vi "Setup.vi"(4 "Exit on Error / V / H (T)":bool=TRUE, 5 "Description":string, 6 "Arguments (From Args)":string[](array[string]), 7 "Name":string, 8 "error in (no error)":errorcluster, 9 "Version":string, 11 "Arguments":T1[](array[typedef]) {"Number" items=["? One or none"=0, "* Any"=-1, "+ At least one"=-2]}) -> (0 "error out":errorcluster, 2 "Output":string, 3 "LV Argument Parser out":refnum<class "LV Argument Parser.lvclass">)   [LabVIEW 2020, in "LV ArgParse.lvlib" / "LV Argument Parser.lvclass"]
uses:
  LV Argument Parser.lvclass
  Argument Definition.ctl
  Program Info.ctl
  LV Argument Parser.lvclass/LV Argument Parser.ctl
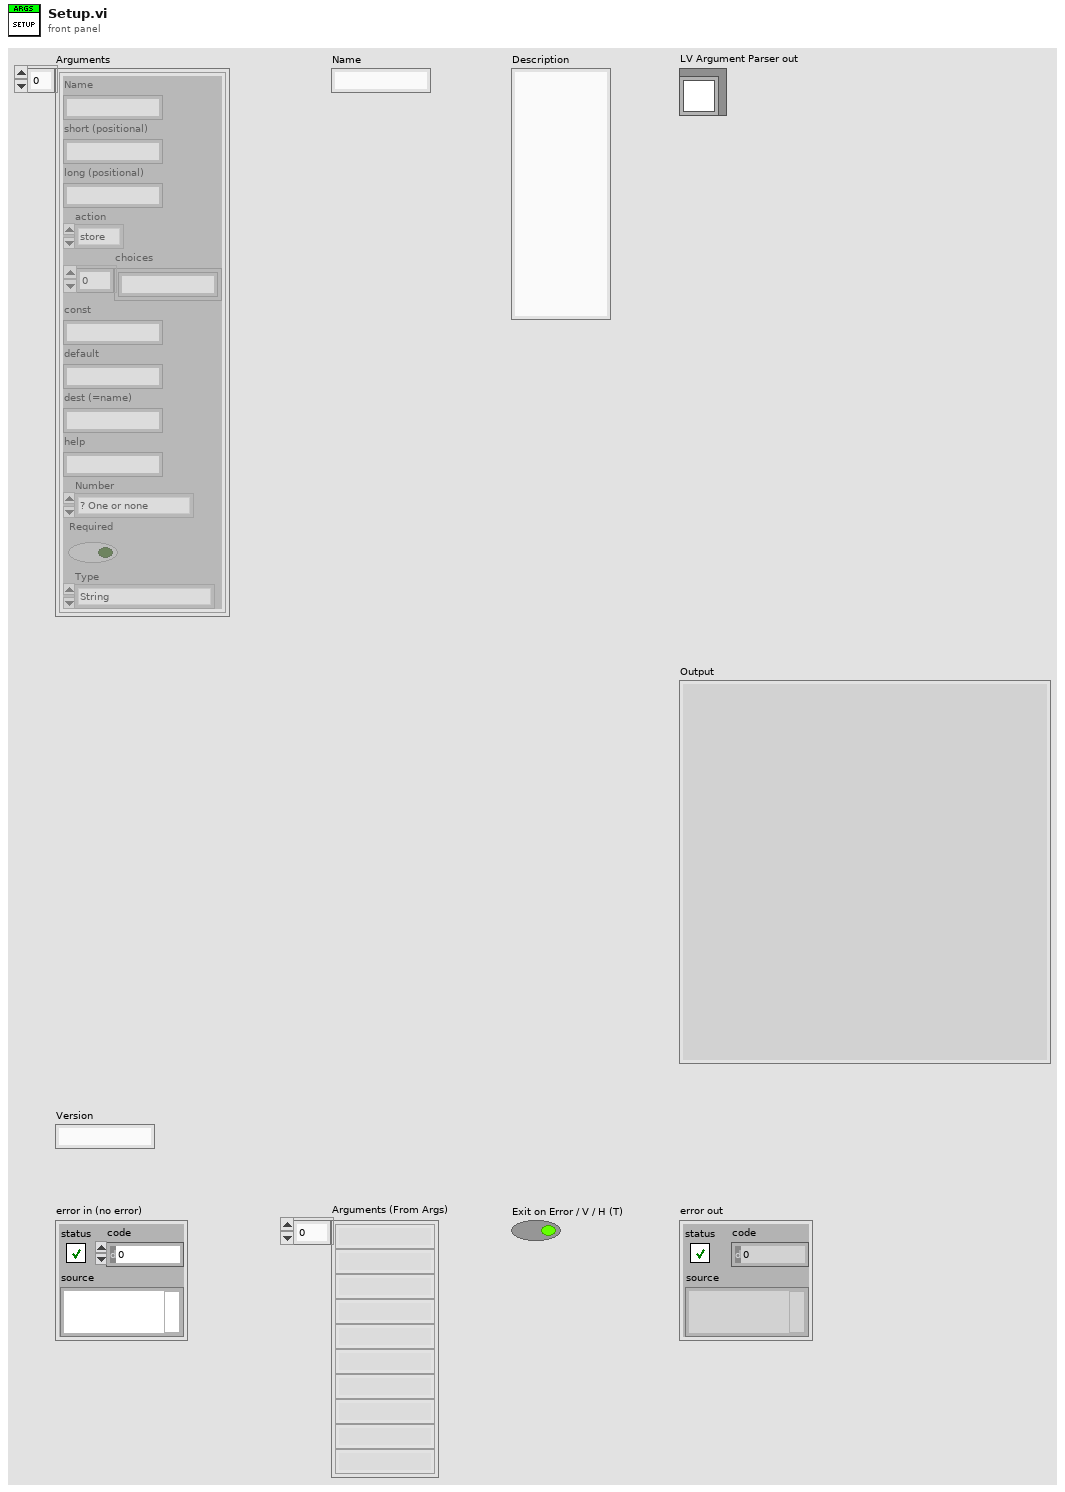
[diagram p1: front panel]
types:
  T1 = typedef "LV ArgParse.lvlib/LV Argument Parser.lvclass/Argument Definition.ctl" = cluster{"Name":string, "short (positional)":string, "long (positional)":string, "action":enum16{"store", "store-const", "store-false", "store-true", "append", "append-const", "count", "help", "version"}, "choices":string[], "const":string, "default":string, "dest (=name)":string, "help":string, "Number":i32, "Required":bool, "Type":enum16{"String", "Int", "UInt", "Float", "Bool", "Date", "Path"}}
  T2 = typedef "LV ArgParse.lvlib/LV Argument Parser.lvclass/Program Info.ctl" = cluster{"Name":string, "Description":string, "Version":string}
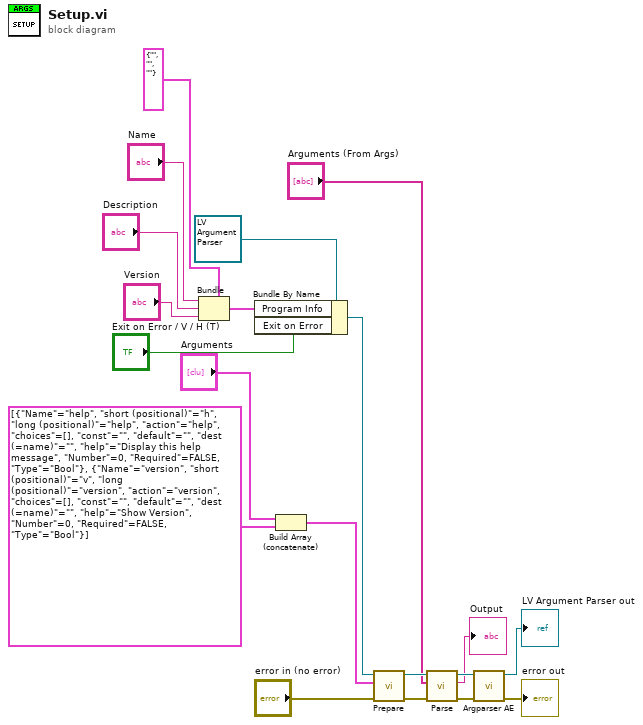
[diagram p0: block diagram]
diagram:
  n1 = Bundle(cluster=T2 {"Name"="", "Description"="", "Version"=""} ("Program Info"), "Name"="Name", "Description"="Description", "Version"="Version") -> (w13:T2)
  n2 = Bundle By Name(cluster=refnum<class "LV Argument Parser.lvclass"> refnum ("LV Argument Parser in"), "Program Info"=w13, "Exit on Error"="Exit on Error / V / H (T)") -> (w14:refnum<class "LV Argument Parser.lvclass">)
  n3 = Build Array (concatenate)("Arguments", T1[] [{"Name"="help", "short (positional)"="h", "long (positional)"="help", "action"=enum."help", "choices"=[], "const"="", "default"="", "dest (=name)"="", "help"="Display this help message", "Number"=0, "Required"=FALSE, "Type"=enum."Bool"}, {"Name"="version", "short (positional)"="v", "long (positional)"="version", "action"=enum."version", "choices"=[], "const"="", "default"="", "dest (=name)"="", "help"="Show Version", "Number"=0, "Required"=FALSE, "Type"=enum."Bool"}] ("Array")) -> (w10:T1[])
  n4 = call "Prepare.vi"("error in (no error)"="error in (no error)", "Arguments"=w10, "LV Argument Parser in"=w14) -> ("error out"=w19:errorcluster, "LV Argument Parser out"=w5:refnum<class "LV Argument Parser.lvclass">)  [unwired: 7 in]
  n5 = call "Parse.vi"("error in (no error)"=w19, "Arguments (From Args)"="Arguments (From Args)", "LV Argument Parser in (Global)"=w5) -> ("error out"=w6:errorcluster, "Output"=→"Output":string, "LV Argument Parser out"=w4:refnum<class "LV Argument Parser.lvclass">)  [unwired: 6 in]
  n6 = call "Argparser AE.vi"("error in (no error)"=w6, "LV Argument Parser in"=w4) -> ("error out"=→"error out":errorcluster, "LV Argument Parser out"=→"LV Argument Parser out":refnum<class "LV Argument Parser.lvclass">)  [unwired: 8 in]
